vi "VIH Utility - FILE - List Directory w Exclusion Patterns.vi"(8 "error in":errorcluster, 9 "Exclude patterns":string[](array[string]), 10 "Include patterns":string[](array[string]), 11 "directory path":path) -> (0 "error out":errorcluster, 1 "directory paths":path[](array[path]), 2 "file paths":path[](array[path]), 3 "dup directory path":path)   [LabVIEW 2014]
doc: "::: VI Helpeks :::\nCopyright (c) 2000-2026 Konstantin Shifershteyn. All rights reserved."
panel:
  # "VI Helpeks\nCopyright (c) 2012-2026 Konstantin Shifershteyn"
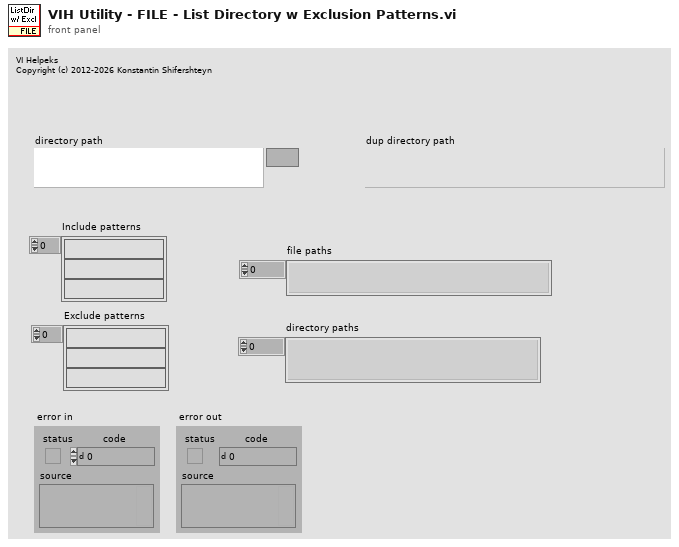
[diagram p1: front panel]
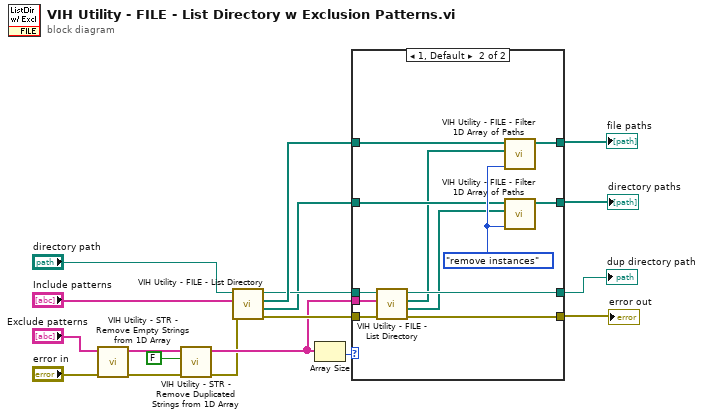
[diagram p0: block diagram]
diagram:
  n1 = call "VIH Utility - STR - Remove Empty Strings from 1D Array.vi"("error in"="error in", "String array in"="Exclude patterns") -> ("error out"=w4:errorcluster, "String array out"=w10:string[])  [unwired: 8 in]
  n2 = call "VIH Utility - STR - Remove Duplicated Strings from 1D Array.vi"("error in (no error)"=w4, "case sensitive comparison (T)"=FALSE, "Array in"=w10) -> ("error out"=w5:errorcluster, "Array out"=w8:string[])  [unwired: 7 in]
  n3 = call "VIH Utility - FILE - List Directory.vi"("error in"=w5, "patterns"="Include patterns", "directory path"="directory path") -> ("error out"=w16:errorcluster, "directory paths"=w14:path[], "file paths"=w18:path[], "dup directory path"=w17:path)  [unwired: 5 out]
  n4 = Array Size(array=w8) -> (size(s)=w11:i32)
  n5 = case shown="1, Default" w11 {
    tunnel: [w22 w34] -> w2
    tunnel: w18 -> [w22 w26]
    tunnel: w17 -> [w20 w33]
    tunnel: w16 -> [w19 w32]
    tunnel: w8 -> [_ w31]
    tunnel: w14 -> [w21 w25]
    tunnel: [w20 w30] -> w13
    tunnel: [w19 w29] -> w12
    tunnel: [w21 w28] -> w3
    frame 0 {
    }
    frame 1, Default {
      w27 = enum16{"keep instances", "remove instances"}."remove instances" ("Action")
      n6 = call "VIH Utility - FILE - List Directory.vi"("error in"=w32, "patterns"=w31, "directory path"=w33) -> ("error out"=w29:errorcluster, "directory paths"=w23:path[], "file paths"=w24:path[], "dup directory path"=w30:path)  [unwired: 5 out]
      n7 = call "VIH Utility - FILE - Filter 1D Array of Paths.vi"("Action (keep instances)"=w27, "Instances"=w24, "Paths in"=w26) -> ("Paths out"=w34:path[])  [unwired: 4 in]
      n8 = call "VIH Utility - FILE - Filter 1D Array of Paths.vi"("Action (keep instances)"=w27, "Instances"=w23, "Paths in"=w25) -> ("Paths out"=w28:path[])  [unwired: 4 in]
    }
  }
  "error out" <- w12
  "directory paths" <- w3
  "dup directory path" <- w13
  "file paths" <- w2
